vi "_Parse Markdown Note Elements.vi"(8 "Error in":errorcluster caption="Error in (no error)", 11 "Lines":string[](array[string])) -> (0 "Error out":errorcluster, 2 "Array":T1[](array[typedef]), 3 "Lines (dup)":string[](array[string]))   [LabVIEW 2017, in "csmdoc.lvlib"]
uses:
  csmdoc.lvlib
  _Typedef/DocNote.ctl
  _tool/_file/csm-file-support.lvlib
  Communicable State Machine.lvlib
  _Shared/CSM Shared.lvlib
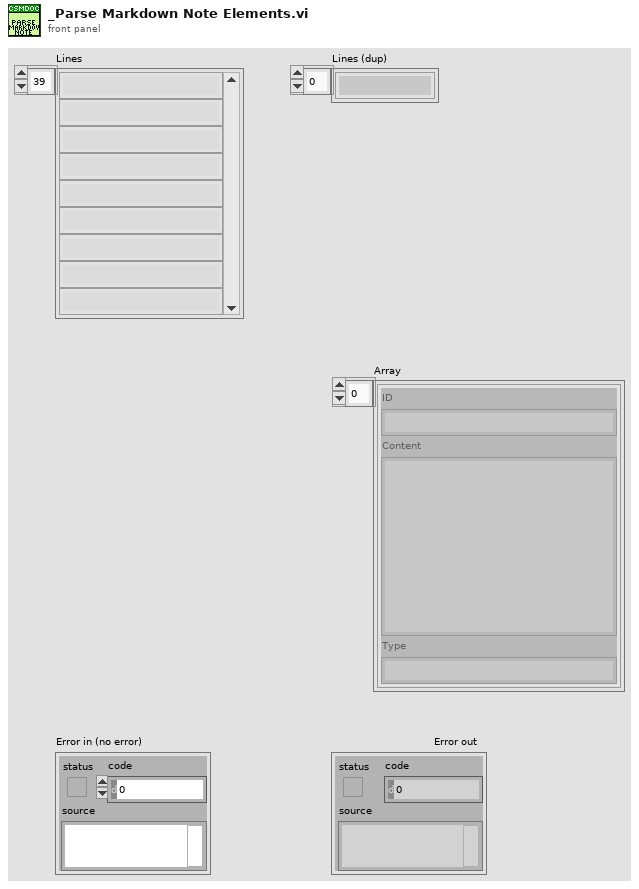
[diagram p1: front panel]
types:
  T1 = typedef "csmdoc.lvlib/DocNote.ctl" = cluster{"ID":string, "Content":string, "Type":string}
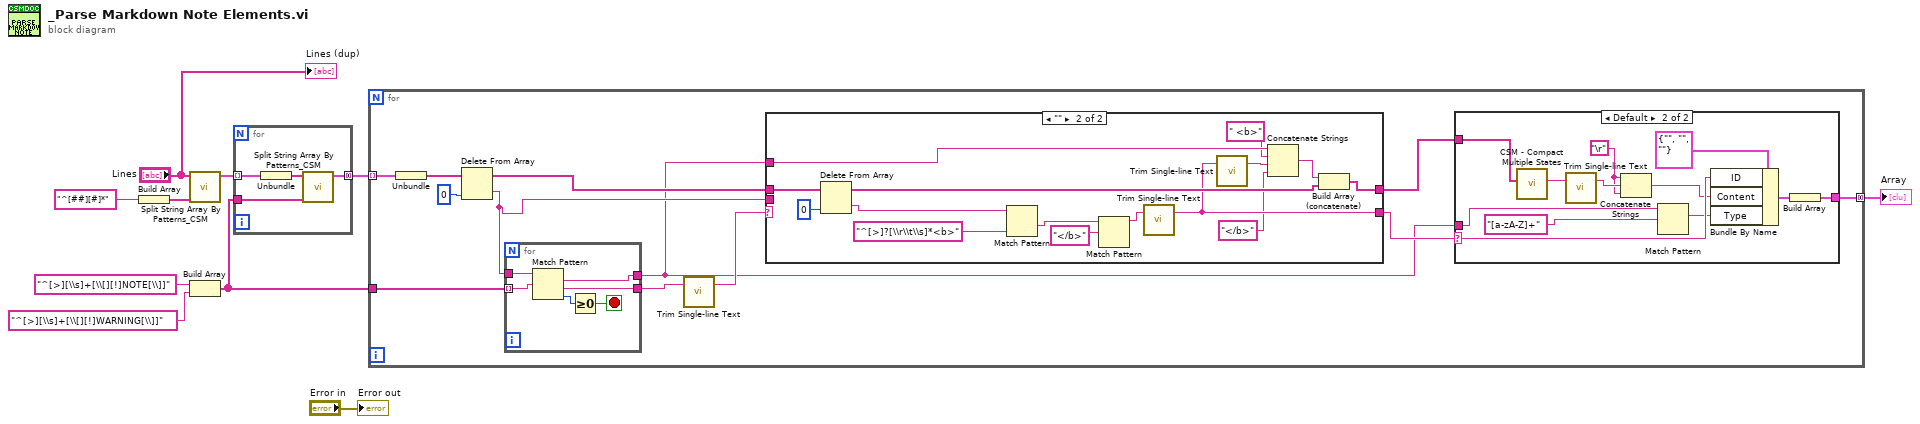
[diagram p0: block diagram]
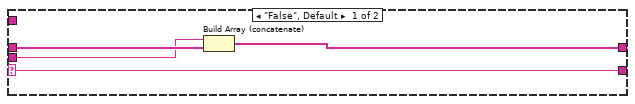
[diagram p2: hidden frame]
diagram:
  n1 = Build Array("^[##][#]*" ("delimited string")) -> (w4:string[])
  n2 = call "Split String Array By Patterns_CSM.vi"("Patterns"=w4, "Text Array"="Lines") -> ("Array"=w5:cluster{"filtered array":string[]}[])  [unwired: 9 in]
  n3 = Build Array("^[>][\\s]+[\\[][!]NOTE[\\]]" ("delimited string"), "^[>][\\s]+[\\[][!]WARNING[\\]]" ("delimited string")) -> (w9:string[])
  n4 = for {
    tunnel: w5 -> [w14] mode=indexing
    tunnel: [w12] -> w6 mode=concatenating
    tunnel: w9 -> [w11]
    n5 = Unbundle(w14) -> ("filtered array"=w13:string[])
    n6 = call "Split String Array By Patterns_CSM.vi"("Patterns"=w11, "Text Array"=w13) -> ("Array"=w12:cluster{"filtered array":string[]}[])  [unwired: 9 in]
  }
  n7 = for {
    tunnel: w6 -> [w26] mode=indexing
    tunnel: [w23] -> w10 mode=concatenating
    tunnel: w9 -> [w22]
    n8 = Unbundle(w26) -> ("filtered array"=w21:string[])
    n9 = Delete From Array(array=w21, index=0) -> (deleted portion=w16:string, array with subset deleted=w20:string[])  [unwired: 1 in]
    n10 = for {
      tunnel: w16 -> [w50]
      tunnel: [w51] -> w24
      tunnel: w22 -> [w49] mode=indexing
      tunnel: [w46] -> w15
      stop <- w47 stop-if-true
      n11 = Match Pattern(string=w50, regular expression=w49) -> (match substring=w46:string, after substring=w51:string, offset past match=w48:i32)  [unwired: 1 in, 1 out]
      n12 = Greater Or Equal To 0?(x=w48) -> (x >= 0?=w47:bool)
    }
    n13 = call "Trim Single-line Text.vi"("single-line text"=w24) -> ("trimed text"=w19:string)  [unwired: 2 in]
    n14 = case shown="\"\"" w19 {
      selector: w19 -> [w28 _]
      tunnel: w20 -> [w30 w44]
      tunnel: [w28 w33] -> w18
      tunnel: [w29 w39] -> w17
      tunnel: w16 -> [w27 _]
      tunnel: w15 -> [_ w37]
      frame "False", Default {
        n15 = Build Array (concatenate)(w27, w30) -> (w29:string[])
      }
      frame "" {
        n16 = Delete From Array(array=w44, index=0) -> (deleted portion=w35:string, array with subset deleted=w38:string[])  [unwired: 1 in]
        n17 = Match Pattern(string=w35, regular expression="^[>]?[\\r\\t\\s]*<b>") -> (after substring=w41:string)  [unwired: 1 in, 3 out]
        n18 = Match Pattern(string=w41, regular expression="</b>") -> (before substring=w40:string)  [unwired: 1 in, 3 out]
        n19 = call "Trim Single-line Text.vi"("single-line text"=w40) -> ("trimed text"=w33:string)  [unwired: 2 in]
        n20 = call "Trim Single-line Text.vi"("single-line text"=w33) -> ("trimed text"=w34:string)  [unwired: 2 in]
        n21 = Concatenate Strings(w37, " <b>" ("string"), w34, "</b>" ("string")) -> (w36:string)
        n22 = Build Array (concatenate)(w36, w38) -> (w39:string[])
      }
    }
    n23 = case shown="Default" w18 {
      selector: w18 -> [_ w62]
      tunnel: [_ w59] -> w23
      tunnel: w15 -> [_ w57]
      tunnel: w17 -> [_ w55]
      frame "" {
      }
      frame Default {
        w52 = "\r"
        n24 = call "CSM - Compact Multiple States.vi"("Multiple States"=w55) -> ("States"=w61:string)  [unwired: 9 in]
        n25 = call "Trim Single-line Text.vi"("single-line text"=w61) -> ("trimed text"=w54:string)  [unwired: 2 in]
        n26 = Concatenate Strings(w52, w54, w52) -> (w53:string)
        n27 = Match Pattern(string=w57, regular expression="[a-zA-Z]+") -> (match substring=w56:string)  [unwired: 1 in, 3 out]
        n28 = Bundle By Name(cluster=T1 {"ID"="", "Content"="", "Type"=""} ("Cluster"), "ID"=w62, "Content"=w53, "Type"=w56) -> (w60:T1)
        n29 = Build Array(w60) -> (w59:T1[])
      }
    }
  }
  "Array" <- w10
  "Error out" <- "Error in"
  "Lines (dup)" <- "Lines"
